vi "Delete_User_in_program.vi"(8 "error in (no error)":errorcluster) -> (0 "error out":errorcluster)   [LabVIEW 2021]
panel:
  in  "Back Button":bool
  in  "Remove user":bool
  out "Result":bool
  out "element":string
  out "Ring - Menu 2":u16(ring)
  in  "Ring - Menu":u16(ring)
  in  "Multicolumn Listbox":i32(listbox)
  out "array w/ subset deleted":string[](array[string])
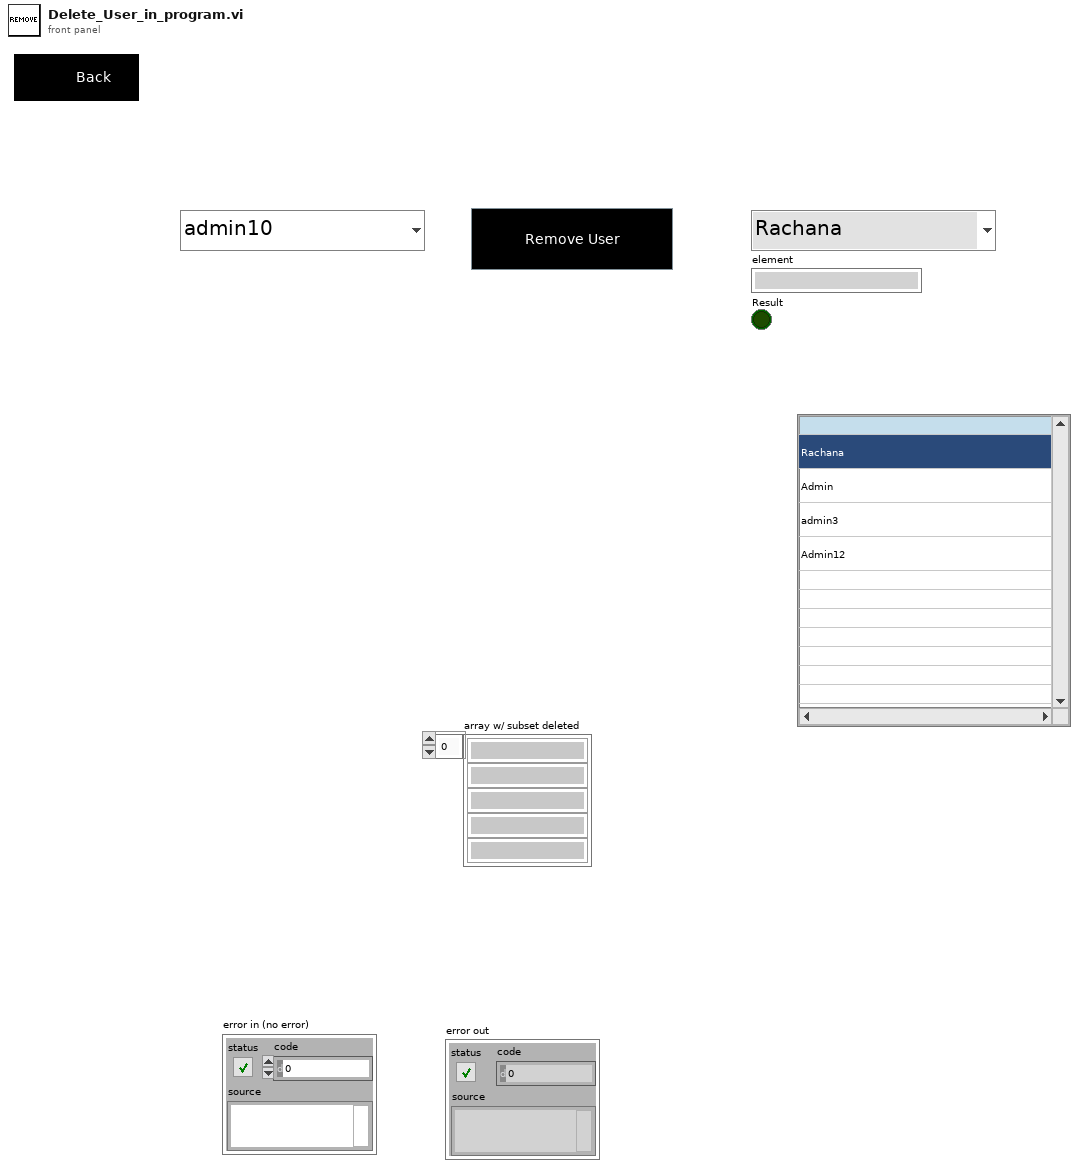
[diagram p1: front panel]
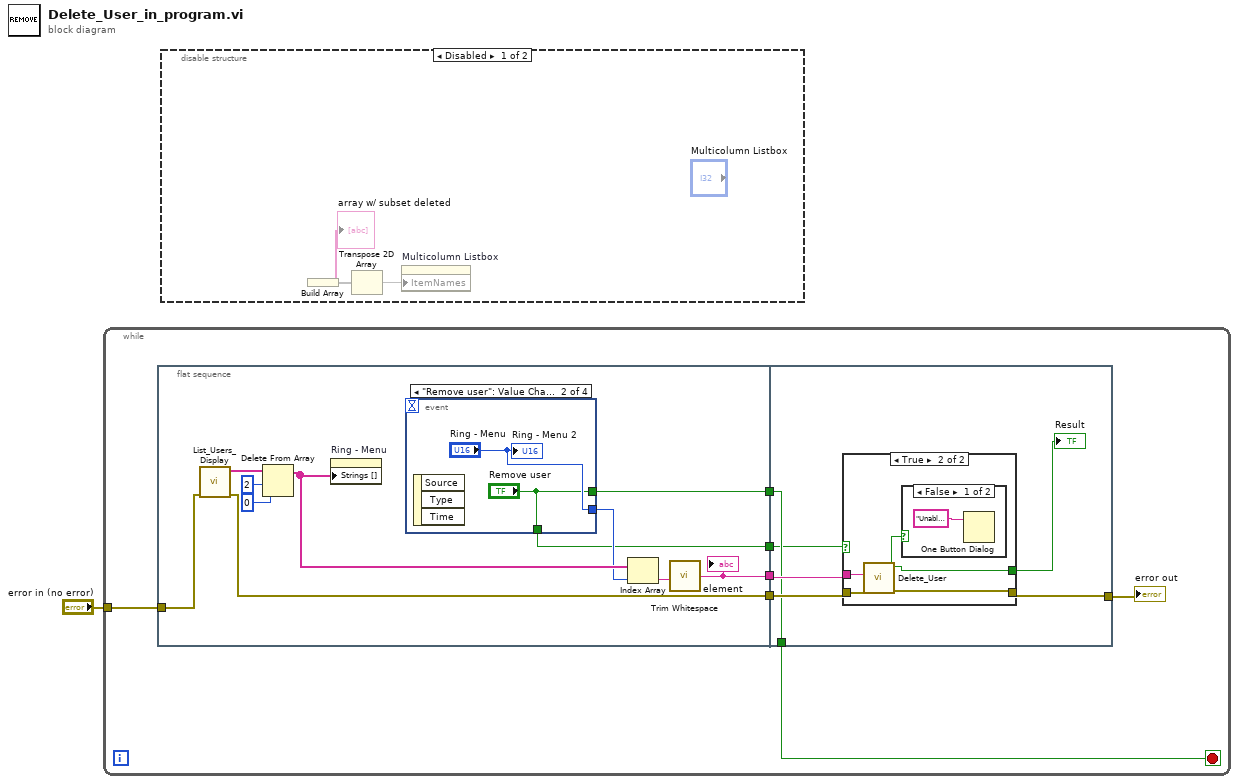
[diagram p0: block diagram]
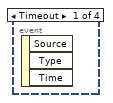
[diagram p2: hidden frame]
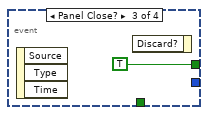
[diagram p3: hidden frame]
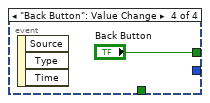
[diagram p4: hidden frame]
diagram:
  n1 = while {
    tunnel: "error in (no error)" -> [w6]
    stop <- w3 stop-if-true
    n2 = flat-sequence {
      tunnel: [w14] -> w8
      tunnel: w6 -> [w12]
      tunnel: [w11] -> w7
      tunnel: [w10] -> w4
      tunnel: [w9] -> w2
      tunnel: w8 -> [w29]
      tunnel: w7 -> [w28]
      tunnel: [w27] -> w5
      tunnel: w4 -> [w26]
      tunnel: [w26] -> w3
      tunnel: w2 -> [w25]
      frame #0 {
        n3 = call "List_Users_Display.vi"("error in (no error)"=w12) -> ("error out"=w11:errorcluster, "Array"=w19:string[])  [unwired: 9 in]
        n4 = Delete From Array(array=w19, length=2, index=0) -> (array with subset deleted=w16:string[])  [unwired: 1 out]
        n5 = property on="Ring - Menu" class="Ring (strict)"("Strings []"=w16) -> ()  [unwired: 2 in, 2 out]
        n6 = event shown="[1] \"Remove user\": Value Change" {
          selector: _ -> [_ _ _ _]
          dyn-events: _ -> [_ _ _ _]
          timeout: _ -> [_ _ _ _]
          tunnel: [_ "Ring - Menu" _ _] -> w13
          tunnel: [_ "Remove user" TRUE "Back Button"] -> w10
          tunnel: [_ "Remove user" _ _] -> w9
          event Timeout {
            n7 = event-data() -> ()  [unwired: 1 in, 3 out]
          }
          event "Remove user": Value Change {
            n8 = event-data() -> ()  [unwired: 1 in, 3 out]
            "Ring - Menu 2" <- "Ring - Menu"
          }
          event Panel Close? {
            n9 = event-data() -> ()  [unwired: 1 in, 3 out]
            n10 = event-data() -> ()  [unwired: 2 in, 1 out]
          }
          event "Back Button": Value Change {
            n11 = event-data() -> ()  [unwired: 1 in, 3 out]
          }
        }
        n12 = Index Array(array=w16, index=w13) -> (element=w15:string)
        n13 = call <vilib>:"Trim Whitespace.vi"("string"=w15) -> ("trimmed string"=w14:string)  [unwired: 1 in]
        "element" <- w14
      }
      frame #1 {
        n14 = case shown="True" w25 {
          tunnel: w29 -> [_ w34]
          tunnel: [_ w33] -> w24
          tunnel: w28 -> [w30 w32]
          tunnel: [w30 w31] -> w27
          frame False {
          }
          frame True {
            n15 = call "Delete_User.vi"("error in (no error)"=w32, "Name"=w34) -> ("error out"=w31:errorcluster, "Result"=w33:bool)  [unwired: 8 in]
            n16 = case shown="False" w33 {
              frame False {
                n17 = One Button Dialog(message="Unable to remove the user") -> ()  [unwired: 1 in, 1 out]
              }
              frame True {
              }
            }
          }
        }
        "Result" <- w24
      }
    }
    "error out" <- w5
  }
  n18 = disable-structure shown="Disabled" {
    frame Disabled {
      n19 = Build Array("array w/ subset deleted") -> (w36:void[])
      n20 = Transpose 2D Array(2D array=w36) -> (transposed array=w37:void[][])
      n21 = property on="Multicolumn Listbox" class="MCListbox (strict)"("ItemNames"=w37) -> ()  [unwired: 2 in, 2 out]
    }
    frame Enabled {
    }
  }
